vi "Configure Session.vi"(8 "error in":errorcluster, 11 "Plugin in":refnum<class "Nominal-Streamer.lvclass">) -> (0 "error out":errorcluster, 3 "Plugin out":refnum<class "Nominal-Streamer.lvclass">)   [LabVIEW 2020, in "Nominal-Streamer.lvlib" / "Nominal-Streamer.lvclass"]
uses:
  Nominal-Streamer.lvclass
  Nominal-Streamer.lvclass/Nominal-Streamer.ctl
  async stream processor.vi
  <vilib>/FlexLogger/SDK/PluginSDK.lvlibp/PEFClasses/SDK/Channel/Channel.lvclass
  <vilib>/FlexLogger/SDK/PluginSDK.lvlibp/PEFClasses/SDK/Plugin/Plugin.lvclass
  async queue data.ctl
  <vilib>/FlexLogger/SDK/PluginSDK.lvlibp/PEFClasses/SDK/Plugin/ParameterAccess/Read String.vi
  <vilib>/Utility/SystemLogging/NI_SystemLogging.lvlib
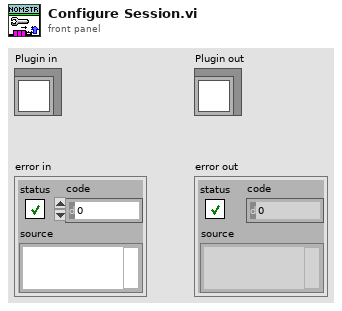
[diagram p1: front panel]
types:
  T1 = typedef "Nominal-Streamer.lvlib/Nominal-Streamer.lvclass/async queue data.ctl" = cluster{"data values":waveform(dbl)[], "data names":string[]}
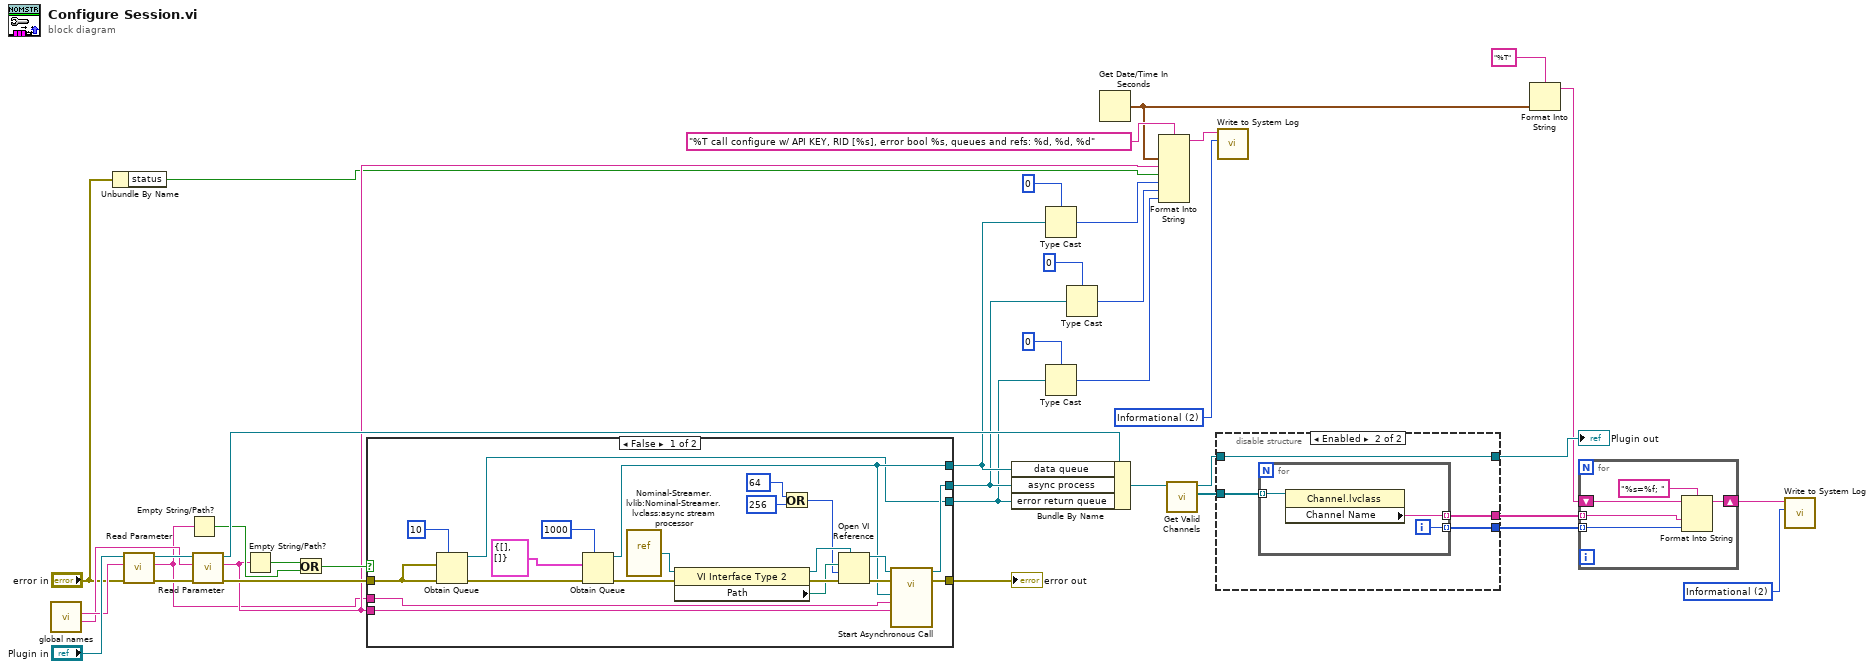
[diagram p0: block diagram]
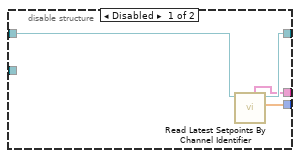
[diagram p2: hidden frame]
diagram:
  w8 = 2 items=["Error", "Warning", "Informational"] ("severity")
  w10 = 2 items=["Error", "Warning", "Informational"] ("severity")
  n1 = call "global names.vi"() -> ("dataset RID"=w32:string, "API Key"=w33:string)  [unwired: 9 in, 1 out]
  n2 = Unbundle By Name("error in") -> ("status"=w23:bool)
  n3 = call-poly <vilib>:"Read Parameter.vi"("error in (no error)"="error in", "Name"=w33, "Plugin in"="Plugin in") -> ("error out"=w35:errorcluster, "Value"=w25:string, "Plugin out"=w38:refnum<class "Nominal-Streamer.lvclass">)  [unwired: 5 in, 1 out]
  n4 = Empty String/Path?(string/path=w25) -> (empty?=w29:bool)
  n5 = call-poly <vilib>:"Read Parameter.vi"("error in (no error)"=w35, "Name"=w32, "Plugin in"=w38) -> ("error out"=w34:errorcluster, "Value"=w26:string, "Plugin out"=w36:refnum<class "Nominal-Streamer.lvclass">)  [unwired: 5 in, 1 out]
  n6 = Empty String/Path?(string/path=w26) -> (empty?=w30:bool)
  n7 = Or(x=w30, y=w29) -> (x .or. y?=w28:bool)
  n8 = case shown="False" w28 {
    tunnel: w34 -> [w41 w60]
    tunnel: [w50 w60] -> w31
    tunnel: [w46 _] -> w19
    tunnel: [w45 _] -> w18
    tunnel: w26 -> [w44 _]
    tunnel: w25 -> [w43 _]
    tunnel: [w40 _] -> w17
    frame False {
      n9 = Obtain Queue(max queue size (-1, unlimited)=10, element data type=w41, error in (no error)=w41) -> (queue out=w40:refnum<queue>, error out=w42:errorcluster)  [unwired: 2 in, 1 out]
      n10 = Obtain Queue(max queue size (-1, unlimited)=1000, element data type=T1 {"data values"=[], "data names"=[]} ("Waveform"), error in (no error)=w42) -> (queue out=w46:refnum<queue>, error out=w51:errorcluster)  [unwired: 2 in, 1 out]
      n11 = vi-ref "Nominal-Streamer.lvlib:Nominal-Streamer.lvclass:async stream processor.vi"() -> (w59:refnum<vi>)
      n12 = property class="VI Interface Type 2"(reference=w59, error in=w51) -> (reference out=w56:refnum<vi>, error out=w58:errorcluster, "Path"=w57:path)
      n13 = Or(x=64 ("options"), y=256 ("options")) -> (x .or. y?=w48:i32)
      n14 = Open VI Reference(type specifier VI Refnum (for type only)=w56, vi path=w57, options=w48, error in (no error)=w58) -> (vi reference=w52:refnum<vi>, error out=w53:errorcluster)  [unwired: 2 in]
      n15 = call-by-ref "Start Asynchronous Call"(reference=w52, error in=w53, "dataset RID"=w44, "api key"=w43, "data queue"=w46) -> (reference out=w45:refnum<vi>, error out=w50:errorcluster)  [unwired: 8 in, 1 out]
    }
    frame True {
    }
  }
  "error out" <- w31
  n16 = Bundle By Name(cluster=w36, "data queue"=w19, "async process"=w18, "error return queue"=w17) -> (w4:refnum<class "Nominal-Streamer.lvclass">)
  n17 = Type Cast(type=u32 0, x=w19) -> (*(type *) &x=w15:u32)
  n18 = Type Cast(type=u32 0, x=w17) -> (*(type *) &x=w14:u32)
  n19 = Type Cast(type=u32 0, x=w18) -> (*(type *) &x=w16:u32)
  n20 = Get Date/Time In Seconds() -> (seconds since 1Jan1904=w1:timestamp)
  n21 = Format Into String(format string="%T call configure w/ API KEY, RID [%s], error bool %s, queues and refs: %d, %d, %d", w1, w26, w23, w15, w16, w14) -> (resulting string=w9:string)  [unwired: 2 in, 1 out]
  n22 = call <vilib>:"Get Valid Channels.vi"("Plugin in"=w4) -> ("Channels"=w2:refnum<class "Channel.lvclass">[], "Plugin out"=w3:refnum<class "Nominal-Streamer.lvclass">)  [unwired: 8 in, 1 out]
  n23 = disable-structure shown="Enabled" {
    disable-tunnel: [w64 w68] -> w13
    disable-tunnel: [w63 w65] -> w12
    disable-tunnel: [w62 w66] -> w11
    disable-tunnel: w3 -> [w61 w68]
    disable-tunnel: w2 -> [_ w67]
    frame Disabled {
      n24 = call <vilib>:"Read Latest Setpoints By Channel Identifier.vi"("Plugin in"=w61) -> ("Channel Setpoints"=w63:dbl[], "Plugin out"=w64:refnum<class "Nominal-Streamer.lvclass">, "Names"=w62:string[])  [unwired: 7 in, 1 out]
    }
    frame Enabled {
      n25 = for {
        tunnel: w67 -> [w71] mode=indexing
        tunnel: [w70] -> w66 mode=indexing
        tunnel: [w69] -> w65 mode=indexing
        i -> [w69]
        n26 = property class="Channel.lvclass"(reference=w71) -> ("Channel Name"=w70:string)  [unwired: 1 in, 2 out]
      }
    }
  }
  "Plugin out" <- w13
  n27 = call <vilib>:"Write to System Log.vi"("severity"=w10, "message"=w9) -> ()  [unwired: 9 in, 1 out]
  n28 = Format Into String(format string="%T", w1) -> (resulting string=w6:string)  [unwired: 2 in, 1 out]
  n29 = for {
    tunnel: w12 -> [w76] mode=indexing
    tunnel: w11 -> [w75] mode=indexing
    shift-right: [w74] -> w7
    shift-left: w6 -> [w72]
    n30 = Format Into String(format string="%s=%f; ", initial string=w72, w75, w76) -> (resulting string=w74:string)  [unwired: 1 in, 1 out]
  }
  n31 = call <vilib>:"Write to System Log.vi"("severity"=w8, "message"=w7) -> ()  [unwired: 9 in, 1 out]
